vi "Analog UI Settings.vi"() -> (0 "error out":errorcluster)   [LabVIEW 2021]
uses:
  <userlib>/DAQNavi Polymorphic VI/configure/DAQNavi Get Property/Device/DAQNaviGet_Device_SupportedDevices_Ex.vi
  <vilib>/Utility/config.llb/Write Key (String).vi
  <vilib>/Utility/config.llb/NI_LVConfig.lvlib
panel:
  out "Return message":string
  in  "Button":bool
  in  "Tab Control 2":enum32{"Analog Input", "Analog Output"}(tab)
  in  "AI Channel":string(combo) caption="Channel"
  in  "Device":string(combo) caption="AI Device"
  in  "signal type":string(combo)="Omit"
  in  "value range":string(combo)="Omit"
  in  "Range":string(combo)="Omit"
  in  "AO Device":string(combo)
  in  "Channel":string(combo)
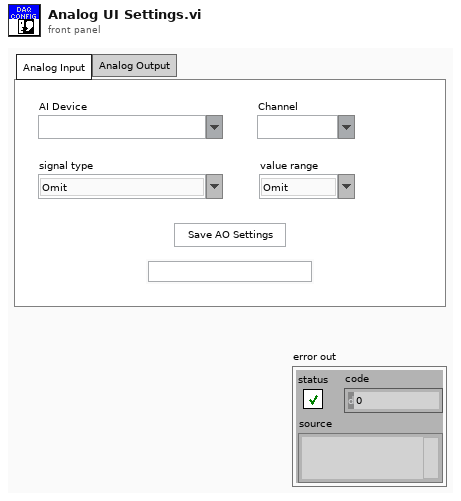
[diagram p1: front panel]
types:
  T1 = enum16{"InstantAi", "BufferedAi", "InstantAo", "BufferedAo", "InstantDi", "InstantDo", "EventCounter", "FreqMeter", "OneShot", "TimerPulse", "PwMeter", "PwModulator", "UdCounter", "WaveformAi"}
  T2 = typedef "NI_LVConfig.lvlib/Config Data RefNum.ctl" = refnum<k1>
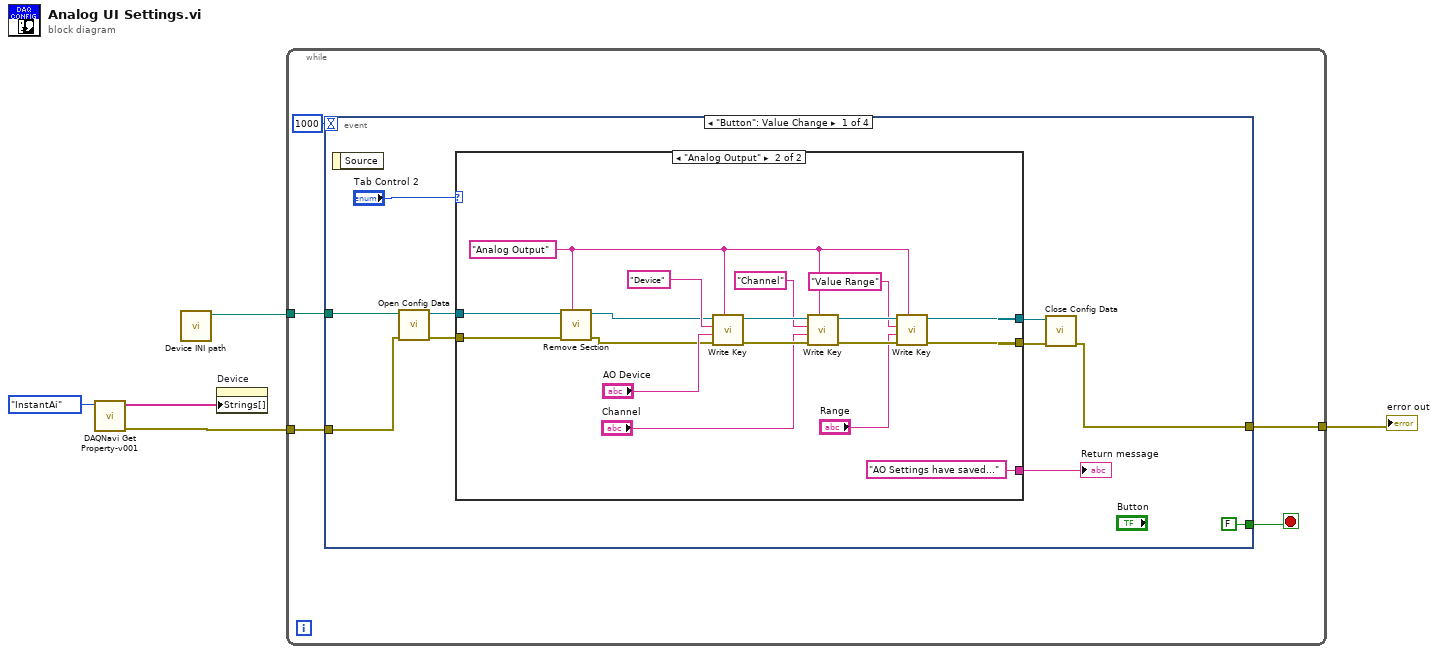
[diagram p0: block diagram]
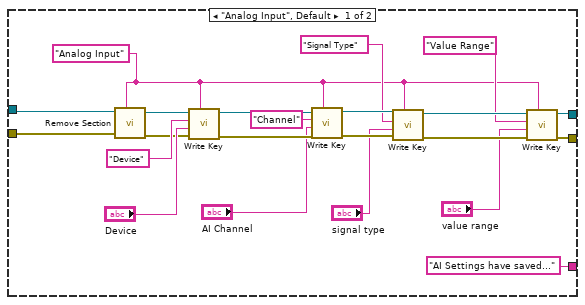
[diagram p2: hidden frame]
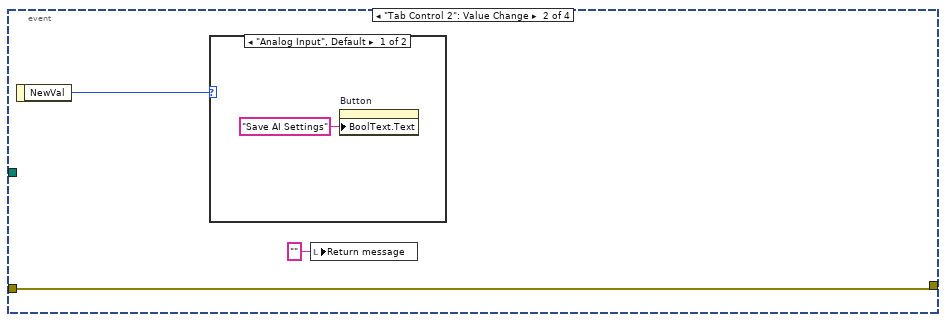
[diagram p3: hidden frame]
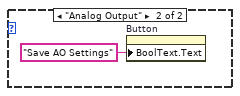
[diagram p4: hidden frame]
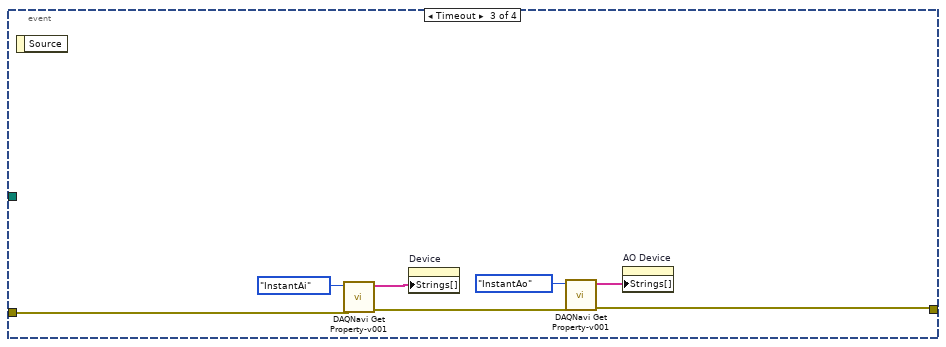
[diagram p5: hidden frame]
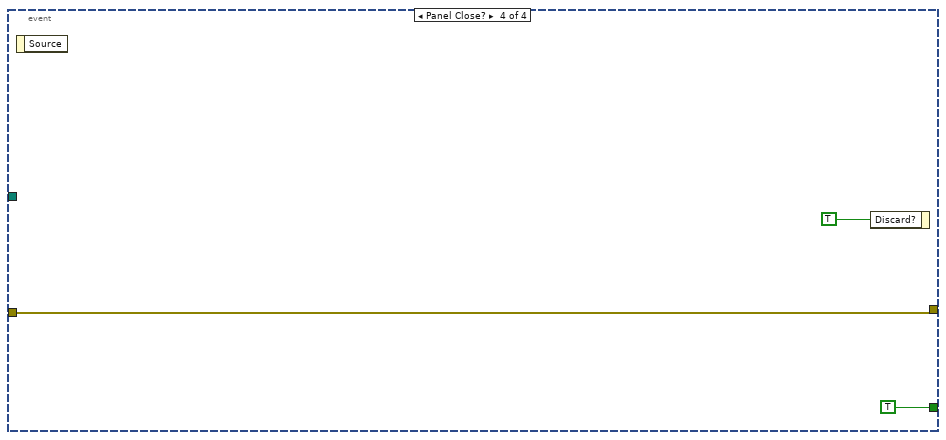
[diagram p6: hidden frame]
diagram:
  n1 = call-poly <userlib>:"DAQNavi Get Property-v001.vi"("DAQNavi Component"=T1."InstantAi") -> ("error out"=w5:errorcluster, "supported devices"=w4:string[])  [unwired: 9 in]
  n2 = call "Device INI path.vi"() -> ("appended path"=w1:path)  [unwired: 11 in]
  n3 = property on="Device" class="CmbBox"("Strings[]"=w4) -> ()  [unwired: 2 in, 2 out]
  n4 = while {
    tunnel: w1 -> [w9]
    tunnel: w5 -> [w8]
    tunnel: [w6] -> w2
    stop <- w10 stop-if-true
    n5 = event shown="[0] \"Button\": Value Change" {
      selector: _ -> [_ _ _ _]
      dyn-events: _ -> [_ _ _ _]
      timeout: 1000 -> [_ _ _ _]
      tunnel: [FALSE ("Button") _ _ TRUE ("Button")] -> w10
      tunnel: w9 -> [w18 _ _ _]
      tunnel: w8 -> [w15 w62 w70 w73]
      tunnel: [w14 w62 w67 w73] -> w6
      event "Button": Value Change {
        n6 = event-data() -> ()  [unwired: 1 in, 1 out]
        n7 = call <vilib>:"Open Config Data.vi"("error in (no error)"=w15, "configuration file path"=w18) -> ("error out"=w20:errorcluster, "refnum"=w19:T2)  [unwired: 7 in, 1 out]
        n8 = case shown="\"Analog Output\"" "Tab Control 2" {
          tunnel: w20 -> [w28 w54]
          tunnel: w19 -> [w25 w52]
          tunnel: [w33 w47] -> w17
          tunnel: [w30 w48] -> w16
          tunnel: ["AI Settings have saved..." "AO Settings have saved..."] -> w12
          frame "Analog Input", Default {
            w22 = "Analog Input" ("key")
            n9 = call <vilib>:"Remove Section.vi"("section"=w22, "error in (no error)"=w28, "refnum"=w25) -> ("error out"=w27:errorcluster, "refnum out"=w26:T2)  [unwired: 6 in, 1 out]
            n10 = call-poly <vilib>:"Write Key.vi"("section"=w22, "error in (no error)"=w27, "value"="Device", "key"="Device", "refnum"=w26) -> ("error out"=w39:errorcluster, "refnum out"=w40:T2)  [unwired: 4 in, 1 out]
            n11 = call-poly <vilib>:"Write Key.vi"("section"=w22, "error in (no error)"=w39, "value"="AI Channel", "key"="Channel", "refnum"=w40) -> ("error out"=w35:errorcluster, "refnum out"=w36:T2)  [unwired: 4 in, 1 out]
            n12 = call-poly <vilib>:"Write Key.vi"("section"=w22, "error in (no error)"=w35, "value"="signal type", "key"="Signal Type", "refnum"=w36) -> ("error out"=w31:errorcluster, "refnum out"=w32:T2)  [unwired: 4 in, 1 out]
            n13 = call-poly <vilib>:"Write Key.vi"("section"=w22, "error in (no error)"=w31, "value"="value range", "key"="Value Range", "refnum"=w32) -> ("error out"=w33:errorcluster, "refnum out"=w30:T2)  [unwired: 4 in, 1 out]
          }
          frame "Analog Output" {
            w44 = "Analog Output" ("section")
            n14 = call <vilib>:"Remove Section.vi"("section"=w44, "error in (no error)"=w54, "refnum"=w52) -> ("error out"=w53:errorcluster, "refnum out"=w51:T2)  [unwired: 6 in, 1 out]
            n15 = call-poly <vilib>:"Write Key.vi"("section"=w44, "error in (no error)"=w53, "value"="AO Device", "key"="Device", "refnum"=w51) -> ("error out"=w59:errorcluster, "refnum out"=w60:T2)  [unwired: 4 in, 1 out]
            n16 = call-poly <vilib>:"Write Key.vi"("section"=w44, "error in (no error)"=w59, "value"="Channel", "key"="Channel", "refnum"=w60) -> ("error out"=w49:errorcluster, "refnum out"=w46:T2)  [unwired: 4 in, 1 out]
            n17 = call-poly <vilib>:"Write Key.vi"("section"=w44, "error in (no error)"=w49, "value"="Range", "key"="Value Range", "refnum"=w46) -> ("error out"=w47:errorcluster, "refnum out"=w48:T2)  [unwired: 4 in, 1 out]
          }
        }
        "Return message" <- w12
        n18 = call <vilib>:"Close Config Data.vi"("error in (no error)"=w17, "refnum"=w16) -> ("error out"=w14:errorcluster)  [unwired: 8 in, 1 out]
      }
      event "Tab Control 2": Value Change {
        n19 = event-data() -> ("NewVal"=w63:enum32{"Analog Input", "Analog Output"})  [unwired: 1 in]
        n20 = case shown="\"Analog Input\", Default" w63 {
          frame "Analog Input", Default {
            n21 = property on="Button" class="Bool"("BoolText.Text"="Save AI Settings" ("Boolean Text.Text")) -> ()  [unwired: 2 in, 2 out]
          }
          frame "Analog Output" {
            n22 = property on="Button" class="Bool"("BoolText.Text"="Save AO Settings" ("Boolean Text.Text")) -> ()  [unwired: 2 in, 2 out]
          }
        }
        n23 = local write "Return message"("" ("Return message")) -> ()
      }
      event Timeout {
        n24 = event-data() -> ()  [unwired: 1 in, 1 out]
        n25 = call-poly <userlib>:"DAQNavi Get Property-v001.vi"("error in (no error)"=w70, "DAQNavi Component"=T1."InstantAi") -> ("error out"=w68:errorcluster, "supported devices"=w71:string[])  [unwired: 8 in]
        n26 = property on="Device" class="CmbBox"("Strings[]"=w71) -> ()  [unwired: 2 in, 2 out]
        n27 = call-poly <userlib>:"DAQNavi Get Property-v001.vi"("error in (no error)"=w68, "DAQNavi Component"=T1."InstantAo") -> ("error out"=w67:errorcluster, "supported devices"=w66:string[])  [unwired: 8 in]
        n28 = property on="AO Device" class="CmbBox"("Strings[]"=w66) -> ()  [unwired: 2 in, 2 out]
      }
      event Panel Close? {
        n29 = event-data() -> ()  [unwired: 1 in, 1 out]
        n30 = event-data("Discard?"=TRUE) -> ()  [unwired: 1 in, 1 out]
      }
    }
  }
  "error out" <- w2
